vi "Load New Bitfile.vi"(7 "Group":bool, 8 "error in (no error)":errorcluster, 10 "NewVal":path, 11 "Item Ref in":T1 format="%.0x") -> (0 "error out":errorcluster, 3 "Section Ref out":T1 format="%.0x")   [LabVIEW 2020, in "FPGA Addon System Explorer.lvlib"]
uses:
  FPGA Addon System Explorer.lvlib
  <vilib>/NI VeriStand/Custom Device API/Custom Device Item Ref.ctl
  Addon Shared/Types/FG Action.ctl
  Addon Shared/SubVIs/Constants.vi
  <vilib>/NI VeriStand/Custom Device Tools/Custom Device Utility Library/NI VeriStand - Search for Item by GUID.vi
  <vilib>/NI/NI VeriStand Advanced SysDef API/SysDef API/SysDef.Property.Get.vi
  <vilib>/NI/NI VeriStand Advanced SysDef API/_SubVIs/SysDef.Property.Get.Variant.vi
  <vilib>/NI/NI VeriStand Advanced SysDef API/SysDef API/SysDef.Property.Set.vi
  <vilib>/NI/NI VeriStand Advanced SysDef API/_SubVIs/SysDef.Property.Set.Variant.vi
  <vilib>/NI VeriStand/Custom Device Tools/Custom Device Utility Library/Custom Device Utility Library.lvlib
  Addon Shared/FPGA Addon Shared.lvlib
  <vilib>/NI VeriStand/Custom Device API/Custom Device API.lvlib
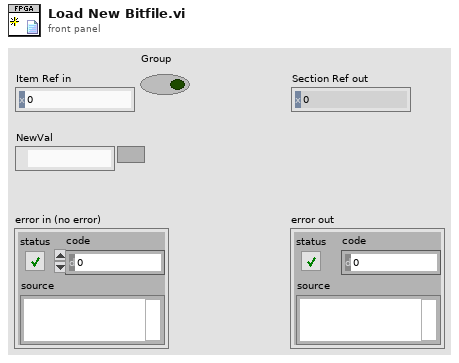
[diagram p1: front panel]
types:
  T1 = typedef "Custom Device API.lvlib/Custom Device Item Ref.ctl" = u64
  T2 = typedef "FPGA Addon Shared.lvlib/FG Action.ctl" = enum8{"GET", "SET"}
  T3 = typedef "Fifo_DMA_Config.ctl" = cluster{"Name":string, "Depth":u32, "Write? (Deprecated:Use Implementation)":bool, "Physical Channel":u32, "Base Address":u32, "Data Width":u32, "Data Type":T4, "FXP Properties":variant, "Write Window Address":u32, "Implementation":T5, "Control Set":u32}
  T4 = typedef "niFpgaDataTypeControl.ctl" = enum32{"Boolean", "I8", "I16", "I32", "I64", "U8", "U16", "U32", "U64", "FXP", "CustomControl", "SGL"}
  T5 = typedef "niFpgaDmaChannelImplementation.ctl" = enum16{"niFpgaTargetToHost", "niFpgaHostToTarget", "niFpgaPeerToPeerWriter", "niFpgaPeerToPeerReader", "niCoreTargetToHost", "niCoreHostToTarget"}
  T6 = typedef "niFpgaBitfileStructure_VI.ctl" = cluster{"Name":string, "RegisterMap":T7[], "Icon":T12}
  T7 = typedef "nirviControlStructure.ctl" = cluster{"Name":string, "Hidden":bool, "Indicator":bool, "Flattened Type":string, "Grouping":cluster{"Grouped":bool, "Member Names":string[], "Member IDs":u32[]}, "Address":u32, "Size":u32, "Class":u32, "Internal":bool, "Typedef":T8, "ID":u32, "Bidirectional":bool, "Synchronous":bool, "Mechanical Action":T9, "Sub Controls":T10[], "Access May Timeout":bool, "Register Node":bool}
  T8 = typedef "nirviTypdefDescription.ctl" = cluster{"Typedef":bool, "Path":path}
  T9 = typedef "nirviMechanicalAction.ctl" = enum8{"Switch When Pressed", "Switch When Released", "Switch Until Released", "Latch When Pressed", "Latch When Released", "Latch Until Released"}
  T10 = typedef "nirviSubControlStructure.ctl" = cluster{"Name":string, "flattened Type":string, "Cluster Information":T11, "Typedef":T8}
  T11 = typedef "nirviClusterElementControl.ctl" = cluster{"Name Hierarchy":string[], "Item Order":u32[]}
  T12 = typedef "imagedata.ctl" = cluster{"image type":i32, "image depth":i32, "image":u8[], "mask":u8[], "colors":u32[], "Rectangle":cluster{"left":i16, "top":i16, "right":i16, "bottom":i16}}
  T13 = typedef "FPGA Addon Shared.lvlib/Register Information.ctl" = cluster{"Name":string, "Data Type":T14, "Default Value":variant, "Attributes":variant}
  T14 = typedef "FPGA Addon Shared.lvlib/FPGA Addon Data Type.ctl" = enum8{"<Null>", "I8", "I16", "I32", "I64", "U8", "U16", "U32", "U64", "SGL", "Boolean", "Analog PWM In Settings", "Analog PWM In", "Digital PWM In Settings", "Digital PWM In", "Digital PWM Out", "Sine Out", "FXP", "FXP+/-24.5", "FXP+/-16.5", "FXP+/-32.8", "FXP+/-64.32", "FXP+/-16.7", "FXP+/-20.5", "FXP+/-27.5", "FXP+/-32.16", "FXP+16.3", "FXP+18.3", "Digital Static In", "Digital Static Out", "Digital Static In Settings", "Digital WSS Out", "Quad Encoder Settings", "Quad Encoder In", "Group"}
  T15 = typedef "FPGA Addon Shared.lvlib/DMA Information.ctl" = cluster{"Name":string, "Data Type":T14}
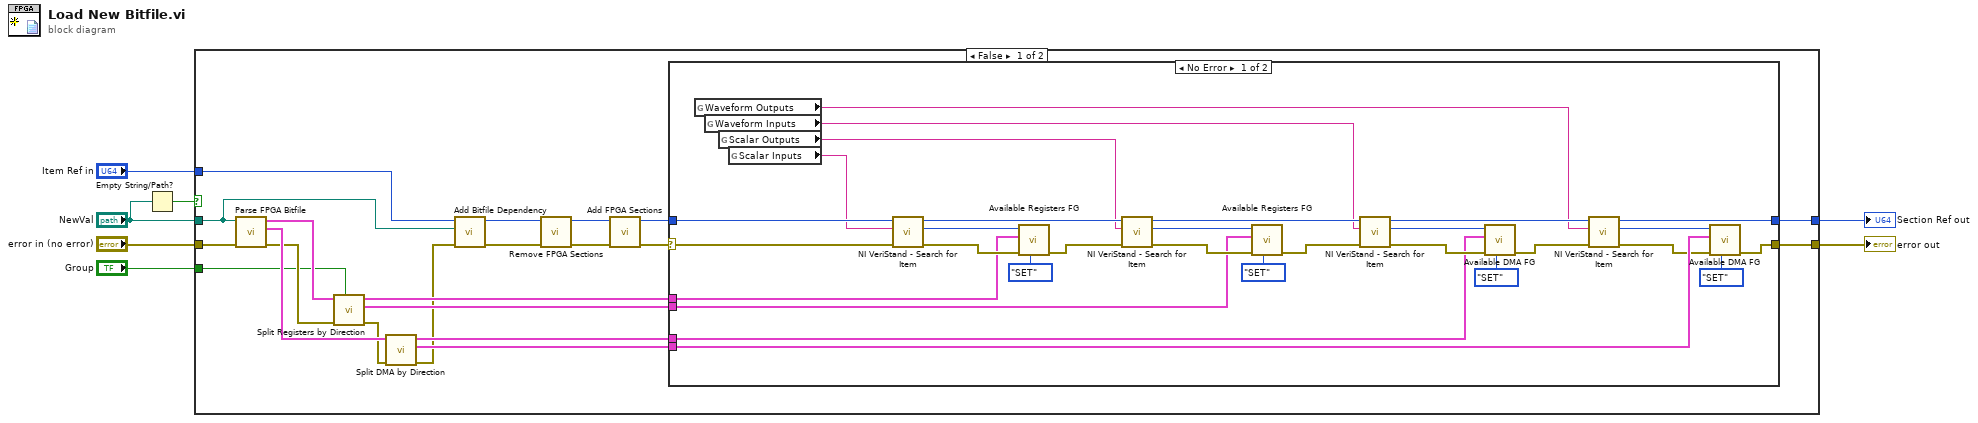
[diagram p0: block diagram]
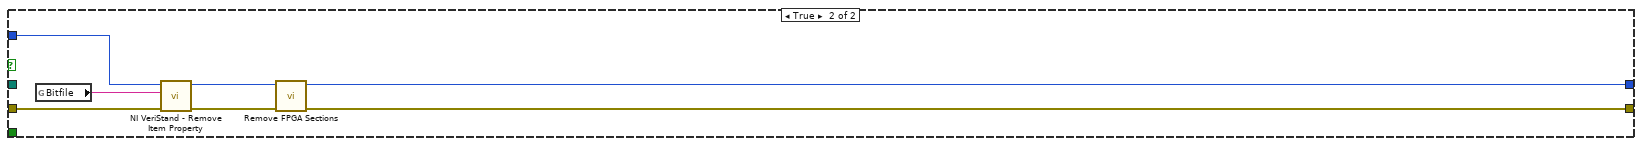
[diagram p3: hidden frame]
diagram:
  n1 = Empty String/Path?(string/path="NewVal") -> (empty?=w5:bool)
  n2 = case shown="False" w5 {
    tunnel: "NewVal" -> [w17 _]
    tunnel: "error in (no error)" -> [w28 w62]
    tunnel: [w22 w67] -> w7
    tunnel: [w21 w66] -> w6
    tunnel: "Item Ref in" -> [w16 w64]
    tunnel: "Group" -> [w9 _]
    frame False {
      n3 = call "Parse FPGA Bitfile.vi"("error in (no error)"=w28, "Path"=w17) -> ("error out"=w12:errorcluster, "DMA configuration array"=w26:T3[], "vi info"=w25:T6)  [unwired: 7 in]
      n4 = call "Split Registers by Direction.vi"("Group"=w9, "error in"=w12, "vi info"=w25) -> ("error out"=w11:errorcluster, "Controls"=w13:T13[], "Indicator"=w14:T13[])  [unwired: 6 in]
      n5 = call "Split DMA by Direction.vi"("error in"=w11, "DMA configuration array"=w26) -> ("error out"=w10:errorcluster, "HostToTarget"=w23:T15[], "TargetToHost"=w24:T15[])  [unwired: 7 in]
      n6 = call "Add Bitfile Dependency.vi"("error in (no error)"=w10, "Path"=w17, "Item Ref in"=w16) -> ("error out"=w18:errorcluster, "Item Ref out"=w15:T1)  [unwired: 6 in, 1 out]
      n7 = call "Remove FPGA Sections.vi"("error in (no error)"=w18, "Item Ref in"=w15) -> ("error out"=w19:errorcluster, "Item Ref out"=w20:T1)  [unwired: 8 in]
      n8 = call "Add FPGA Sections.vi"("error in (no error)"=w19, "Node Ptr"=w20) -> ("error out"=w8:errorcluster, "Parent Ref out"=w27:T1)  [unwired: 8 in]
      n9 = case shown="No Error" w8 {
        selector: w8 -> [w33 w59]
        tunnel: w27 -> [w58 w60]
        tunnel: w24 -> [w45 _]
        tunnel: w23 -> [w40 _]
        tunnel: [w38 w59] -> w22
        tunnel: [w36 w60] -> w21
        tunnel: w14 -> [w35 _]
        tunnel: w13 -> [w34 _]
        frame No Error {
          n10 = global read "Constants.vi" "Waveform Outputs"() -> (w32:string)
          n11 = global read "Constants.vi" "Waveform Inputs"() -> (w31:string)
          n12 = global read "Constants.vi" "Scalar Outputs"() -> (w30:string)
          n13 = global read "Constants.vi" "Scalar Inputs"() -> (w29:string)
          n14 = call-poly <vilib>:"NI VeriStand - Search for Item.vi"("error in"=w33, "Item GUID"=w29, "Section Ref in"=w58) -> ("error out"=w57:errorcluster, "Item Ref"=w56:T1, "Section Ref out"=w54:T1)  [unwired: 5 in, 1 out]
          n15 = call "Available Registers FG.vi"("Action"=FG_Action."SET", "error in (no error)"=w57, "Available Registers"=w35, "Item Ref"=w56) -> ("error out"=w55:errorcluster)  [unwired: 5 in, 2 out]
          n16 = call-poly <vilib>:"NI VeriStand - Search for Item.vi"("error in"=w55, "Item GUID"=w30, "Section Ref in"=w54) -> ("error out"=w49:errorcluster, "Item Ref"=w48:T1, "Section Ref out"=w52:T1)  [unwired: 5 in, 1 out]
          n17 = call "Available Registers FG.vi"("Action"=FG_Action."SET", "error in (no error)"=w49, "Available Registers"=w34, "Item Ref"=w48) -> ("error out"=w47:errorcluster)  [unwired: 5 in, 2 out]
          n18 = call-poly <vilib>:"NI VeriStand - Search for Item.vi"("error in"=w47, "Item GUID"=w31, "Section Ref in"=w52) -> ("error out"=w46:errorcluster, "Item Ref"=w53:T1, "Section Ref out"=w42:T1)  [unwired: 5 in, 1 out]
          n19 = call "Available DMA FG.vi"("Action"=FG_Action."SET", "error in (no error)"=w46, "Available DMA"=w45, "Item Ref"=w53) -> ("error out"=w43:errorcluster)  [unwired: 5 in, 2 out]
          n20 = call-poly <vilib>:"NI VeriStand - Search for Item.vi"("error in"=w43, "Item GUID"=w32, "Section Ref in"=w42) -> ("error out"=w39:errorcluster, "Item Ref"=w41:T1, "Section Ref out"=w36:T1)  [unwired: 5 in, 1 out]
          n21 = call "Available DMA FG.vi"("Action"=FG_Action."SET", "error in (no error)"=w39, "Available DMA"=w40, "Item Ref"=w41) -> ("error out"=w38:errorcluster)  [unwired: 5 in, 2 out]
        }
        frame Error {
        }
      }
    }
    frame True {
      n22 = global read "Constants.vi" "Bitfile"() -> (w65:string)
      n23 = call <vilib>:"NI VeriStand - Remove Item Property.vi"("error in (no error)"=w62, "Property Name"=w65, "Item Ref in"=w64) -> ("error out"=w61:errorcluster, "Item Ref out"=w63:T1)  [unwired: 6 in, 1 out]
      n24 = call "Remove FPGA Sections.vi"("error in (no error)"=w61, "Item Ref in"=w63) -> ("error out"=w67:errorcluster, "Item Ref out"=w66:T1)  [unwired: 8 in]
    }
  }
  "error out" <- w7
  "Section Ref out" <- w6
